vi "P6_SubVIReplace.vi"(11 "Inputs":string[](array[string])) -> (2 "Output/Failure":string, 3 "CLI Process Return Code":i32)   [LabVIEW 2026]
doc: "Slice 1.1 probe: Open VI Reference, Block Diagram, SubVIs[], SubVI Replace with the VI in arg, then read VI Name of SubVIs[0] again."
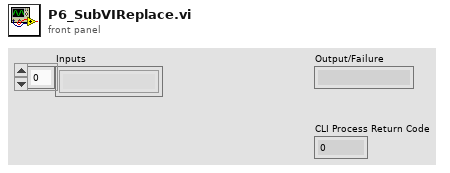
[diagram p1: front panel]
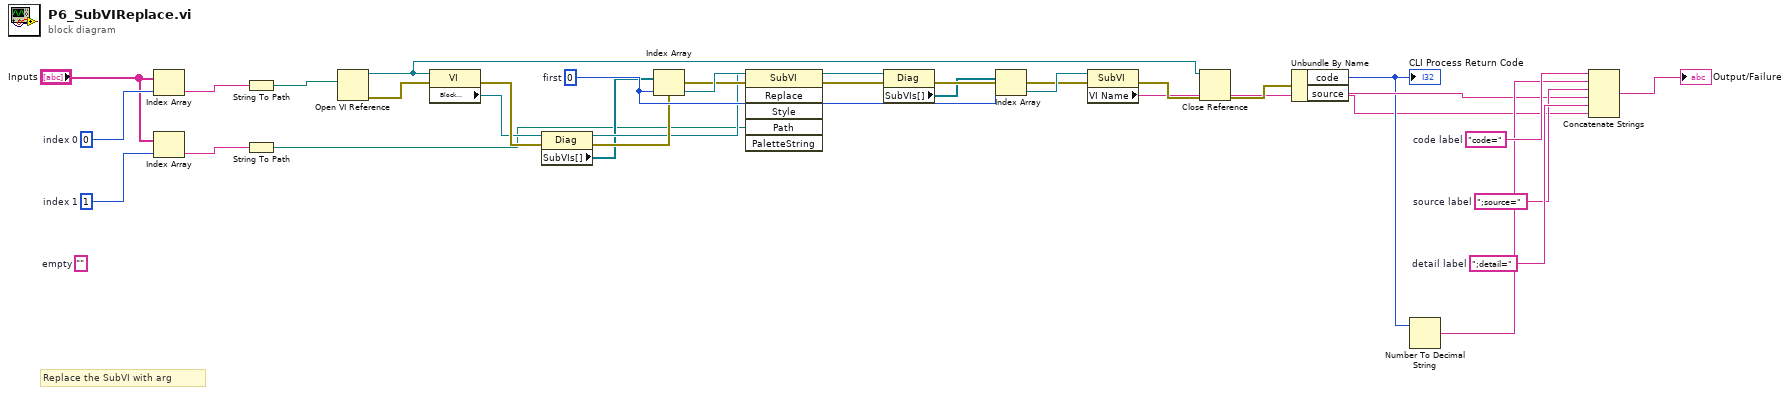
[diagram p0: block diagram]
diagram:
  w29 = ";detail="  # detail label
  w28 = ";source="  # source label
  w27 = "code="  # code label
  w15 = 0  # first
  (unwired) ""  # empty
  w3 = 1  # index 1
  w2 = 0  # index 0
  # "Replace the SubVI with arg"
  n1 = Index Array(array="Inputs", index=w2) -> (element=w4:string)
  n2 = Index Array(array="Inputs", index=w3) -> (element=w5:string)
  n3 = String To Path(string=w4) -> (path=w6:path)
  n4 = String To Path(string=w5) -> (path=w7:path)
  n5 = Open VI Reference(vi path=w6) -> (vi reference=w8:refnum<vi>, error out=w9:errorcluster)  [unwired: 5 in]
  n6 = property class="VI"(reference=w8, error in=w9) -> (error out=w11:errorcluster, "Block Diagram"=w10:refnum<vi>)  [unwired: 1 out]
  n7 = property class="Diag"(reference=w10, error in=w11) -> (reference out=w13:refnum<vi>, error out=w14:errorcluster, "SubVIs[]"=w12:refnum<vi>[])
  n8 = Index Array(array=w12, index=w15) -> (element=w16:refnum<vi>)
  n9 = invoke on="Invoke Node" class="SubVI" method="Replace"(reference=w16, error in=w14, "Path"=w7) -> (error out=w17:errorcluster)  [unwired: 3 in, 5 out]
  n10 = property class="Diag"(reference=w13, error in=w17) -> (error out=w19:errorcluster, "SubVIs[]"=w18:refnum<vi>[])  [unwired: 1 out]
  n11 = Index Array(array=w18, index=w15) -> (element=w20:refnum<vi>)
  n12 = property class="SubVI"(reference=w20, error in=w19) -> (error out=w22:errorcluster, "VI Name"=w21:string)  [unwired: 1 out]
  n13 = Close Reference(reference=w8, error in (no error)=w22) -> (error out=w23:errorcluster)
  n14 = Unbundle By Name(w23) -> ("code"=w24:i32, "source"=w25:string)
  "CLI Process Return Code" <- w24
  n15 = Number To Decimal String(number=w24) -> (decimal integer string=w26:string)  [unwired: 1 in]
  n16 = Concatenate Strings(w27, w26, w28, w25, w29, w21) -> (→"Output/Failure":string)
